vi "Task Stop.vi"(8 "error in (no error)":errorcluster, 11 "SimTask in":refnum<class "SimTask.lvclass">) -> (0 "error out":errorcluster, 3 "SimTask out":refnum<class "SimTask.lvclass">)   [LabVIEW 2020, in "VolatusDemo.lvlib" / "SimTask.lvclass"]
uses:
  SimTask.lvclass
  C:/dev/lv20CE/relink/lv-volatus/Volatus/Task/Task.lvclass
  SimTask.lvclass/SimTask.ctl
  Volatus/Task/Task.lvclass/Task.ctl
  Volatus/Event API/EventAPI.lvclass/EventAPI.ctl
  Volatus/EventHandler Messages/Handle Event Msg/Handle Event Msg.lvclass/Handle Event Msg.ctl
  <vilib>/ActorFramework/Message Enqueuer/Message Enqueuer.lvclass/Message Enqueuer.ctl
  Volatus/Event API/Report Event.vi
  Volatus/EventHandler Messages/Handle Event Msg/Send Handle Event.vi
  <vilib>/ActorFramework/Message Enqueuer/Enqueue.vi
  Volatus/EventHandler Messages/Handle Event Msg/Handle Event Msg.lvclass
  C:/Program Files (x86)/National Instruments/LabVIEW 2020/vi.lib/ActorFramework/Message/Message.lvclass
  Volatus/Task/Task ID.vi
  <vilib>/ActorFramework/Message Priority Queue/Priority Enqueue.vi
  Volatus/Task/Task.lvclass
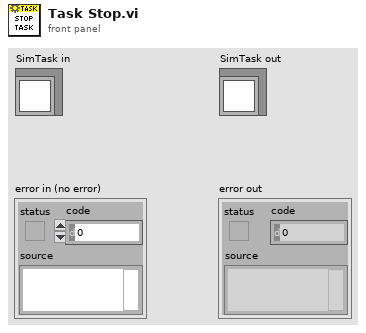
[diagram p1: front panel]
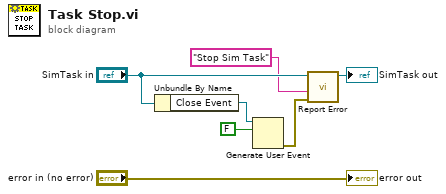
[diagram p0: block diagram]
diagram:
  n1 = Unbundle By Name("SimTask in") -> ("Close Event"=w5:refnum<user-event>)
  n2 = Generate User Event(user event=w5, event data cluster=FALSE ("event data")) -> (error out=w2:errorcluster)  [unwired: 2 in, 1 out]
  n3 = call "Report Error.vi"("error in (no error)"=w2, "Message"="Stop Sim Task" ("Context"), "Task in"="SimTask in") -> ("Task out"=→"SimTask out":refnum<class "SimTask.lvclass">)  [unwired: 7 in, 1 out]
  "error out" <- "error in (no error)"
